vi "query Limit Line Pass Fail.vi"(8 "error in (no error)":errorcluster, 10 "Limit Line Index":i32=1 min=1 max=8, 11 "FSV-40N in":refnum<class "FSV-40N.lvclass">) -> (0 "error out":errorcluster, 2 "Pass?":bool, 3 "FSV-40N out":refnum<class "FSV-40N.lvclass">)   [LabVIEW 2023, in "Spectrum Analyzer.lvlib" / "FSV-40N.lvclass"]
uses:
  FSV-40N.lvclass
  FSV-40N.lvclass/FSV-40N.ctl
  Spectrum Analyzer.lvlib
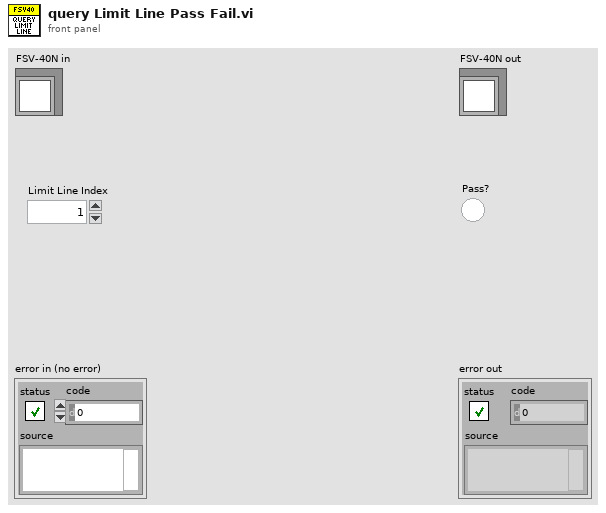
[diagram p1: front panel]
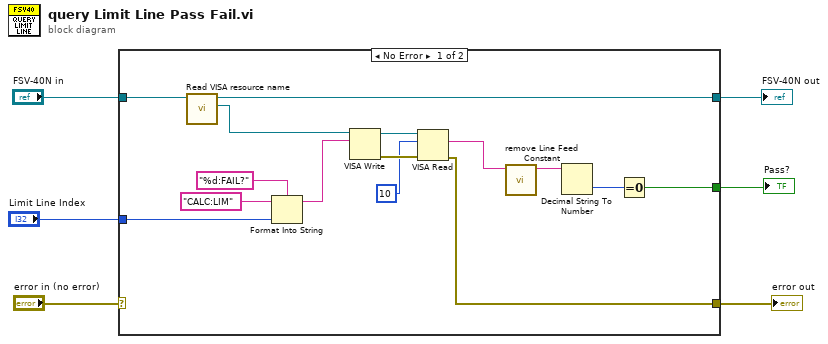
[diagram p0: block diagram]
diagram:
  n1 = case shown="No Error" "error in (no error)" {
    selector: "error in (no error)" -> [_ w22]
    tunnel: "FSV-40N in" -> [w21 w23]
    tunnel: [w17 w23] -> w4
    tunnel: [w7 w22] -> w3
    tunnel: "Limit Line Index" -> [w16 _]
    tunnel: [w8 _] -> w1
    frame No Error {
      n2 = call "Read VISA resource name.vi"("FSV-40N in"=w21) -> ("VISA resource name"=w18:refnum<visa-resource-name>, "FSV-40N out"=w17:refnum<class "FSV-40N.lvclass">)  [unwired: 8 in, 1 out]
      n3 = Format Into String(format string="%d:FAIL?", initial string="CALC:LIM", w16) -> (resulting string=w15:string)  [unwired: 1 in, 1 out]
      n4 = VISA Write(VISA resource name=w18, write buffer=w15) -> (VISA resource name out=w14:refnum<visa-resource-name>, error out=w13:errorcluster)  [unwired: 1 in, 1 out]
      n5 = VISA Read(VISA resource name=w14, byte count=u32 10, error in (no error)=w13) -> (read buffer=w11:string, error out=w7:errorcluster)  [unwired: 2 out]
      n6 = call "remove Line Feed Constant.vi"("Input String"=w11) -> ("Line Feed Removed String"=w10:string)  [unwired: 10 in]
      n7 = Decimal String To Number(string=w10) -> (number=w9:i32)  [unwired: 2 in, 1 out]
      n8 = Equal To 0?(x=w9) -> (x = 0?=w8:bool)
    }
    frame Error {
    }
  }
  "error out" <- w3
  "FSV-40N out" <- w4
  "Pass?" <- w1
